vi "Init+Version.vi"(8 "error in (no error)":errorcluster) -> (0 "error out":errorcluster, 1 "version (str)":string, 2 "minor":i32, 3 "mayor":i32)   [LabVIEW 2020, in "wiringPi.lvlib"]
doc: "<b>_______________________________________________________________</b>\n** Author: Juan José Villacorta\n** LabVIEW wrapper for C library <b> wiringPi </b>,\n** https://github.com/WiringPi/WiringPi\n<b>_______________________________________________________________</b>\n\n\n/*\n * wiringPiSetupGpio:\n * Must be called once at the start of your program execution.\n *\n * GPIO setup: Initialises the system into GPIO Pin mode and uses the\n * memory mapped hardware directly.\n *********************************************************************************\n */"
uses:
  wiringPi.lvlib
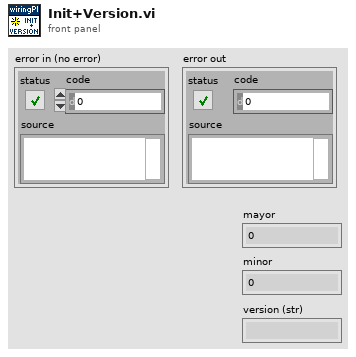
[diagram p1: front panel]
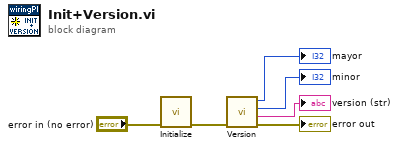
[diagram p0: block diagram]
diagram:
  n1 = call "Initialize.vi"("error in (no error)"="error in (no error)") -> ("error out"=w2:errorcluster)  [unwired: 10 in]
  n2 = call "Version.vi"("error in (no error)"=w2) -> ("error out"=→"error out":errorcluster, "version (str)"=→"version (str)":string, "minor"=→"minor":i32, "mayor"=→"mayor":i32)  [unwired: 7 in]
